vi "vision.vi"() -> ()   [LabVIEW 2024]
uses:
  <vilib>/userDefined/High Color/IMAQdx.ctl
  <vilib>/Python/Open Venv Python Session.vi
  <vilib>/vision/driver/NI_Vision_Acquisition_Software.lvlib
  <vilib>/Instr/_visa.llb/VISA Set IO Buffer Mask.ctl
  <vilib>/Instr/_visa.llb/VISA Flush IO Buffer Mask.ctl
  <vilib>/Instr/_visa.llb/VISA Configure Serial Port (Instr).vi
panel:
  in  "Serial Name":refnum<visa-resource-name>="COM1"
  out "PCU_SPEED (mps)":dbl
  out "PCU_STEER":i16
  out "PCU_ALIVE":u8
  out "하위제어기 통신 패킷":string
  out "RX Data Cnt (byte)":u32
  out "PCU_GEAR":u8
  out "PCU_MODE":u8
  out "ARD_EStop":u8
  out "PCU_ENC":i32
  in  "HLV_AorM":bool
  in  "HLV_SPEED":i16(slide) scale=0.0..1000.0
  out "TX Data Cnt (byte)":u32
  out "string":string
  in  "HLV_GEAR":u8(slide)=1 scale=0.0..2.0
  in  "HLV_EStop":bool
  out "Image":T1(plugin-control)
  in  "Session In":T2
  in  "Lane_No.":i32
  out "ToGoLane_X":dbl[](array[numeric])=[-0.07318960875272751, -0.07601258158683777, -0.07903728634119034, -0.08227015286684036, -0.08571790158748627, -0.08938748389482498, -0.09328625351190567, -0.09742185473442078, -0.1018022671341896, -0.10643591731786728, -0.11133154481649399, -0.11649835854768753, -0.12194599956274033, -0.1276845932006836, -0.13372473418712616, -0.140077605843544, -0.1467549204826355, -0.15376901626586914, -0.1611328274011612, -0.16886006295681, -0.17696507275104523, -0.18546302616596222, -0.19436998665332794, -0.20370280742645264, -0.2134794145822525, -0.22371862828731537, -0.23444052040576935, -0.2456662356853485, -0.2574182152748108, -0.26972031593322754, -0.2825978398323059, -0.2960776686668396, -0.3101884424686432, -0.3249606192111969, -0.3404266834259033, -0.35662132501602173, -0.3735816180706024, -0.39134714007377625, -0.4099603295326233, -0.4294666647911072, -0.44991496205329895, -0.47135770320892334, -0.49385130405426025, -0.5174566507339478, -0.5422393083572388, -0.5682703852653503, -0.5956265330314636, -0.6243910789489746, -0.6546544432640076, -0.6865149736404419]
  out "ToGpLane_Y":dbl[](array[numeric])=[0.040495745837688446, 0.047222185879945755, 0.05409690737724304, 0.06112465262413025, 0.06831060349941254, 0.07565993815660477, 0.08317827433347702, 0.09087134152650833, 0.09874525666236877, 0.10680633038282394, 0.1150611862540245, 0.12351679056882858, 0.13218039274215698, 0.14105971157550812, 0.1501627415418625, 0.159497931599617, 0.16907407343387604, 0.1789005994796753, 0.18898724019527435, 0.19934435188770294, 0.20998279750347137, 0.22091402113437653, 0.23215018212795258, 0.24370405077934265, 0.2555891275405884, 0.2678196132183075, 0.2804107666015625, 0.2933785319328308, 0.306739866733551, 0.3205127418041229, 0.3347163796424866, 0.349371075630188, 0.36449843645095825, 0.38012149930000305, 0.3962647616863251, 0.41295456886291504, 0.43021881580352783, 0.4480874836444855, 0.46659258008003235, 0.48576855659484863, 0.5056522488594055, 0.526283323764801, 0.5477043986320496, 0.5699615478515625, 0.5931042432785034, 0.6171862483024597, 0.6422654986381531, 0.6684049367904663, 0.6956729292869568, 0.7241437435150146]
  out "Tracking_Err(m)":dbl=0.08364582631744388
  in  "Ld(m)":dbl=1.0 format="%#_13g"
  out "GPS_Steer_CMD(Deg)":dbl=-20.0
  out "Lane":T3(graph)=[{"Third_Lane_X"=[-0.07318960875272751, -0.07601258158683777, -0.07903728634119034, -0.08227015286684036, -0.08571790158748627, -0.08938748389482498, -0.09328625351190567, -0.09742185473442078, -0.1018022671341896, -0.10643591731786728, -0.11133154481649399, -0.11649835854768753, -0.12194599956274033, -0.1276845932006836, -0.13372473418712616, -0.140077605843544, -0.1467549204826355, -0.15376901626586914, -0.1611328274011612, -0.16886006295681, -0.17696507275104523, -0.18546302616596222, -0.19436998665332794, -0.20370280742645264, -0.2134794145822525, -0.22371862828731537, -0.23444052040576935, -0.2456662356853485, -0.2574182152748108, -0.26972031593322754, -0.2825978398323059, -0.2960776686668396, -0.3101884424686432, -0.3249606192111969, -0.3404266834259033, -0.35662132501602173, -0.3735816180706024, -0.39134714007377625, -0.4099603295326233, -0.4294666647911072, -0.44991496205329895, -0.47135770320892334, -0.49385130405426025, -0.5174566507339478, -0.5422393083572388, -0.5682703852653503, -0.5956265330314636, -0.6243910789489746, -0.6546544432640076, -0.6865149736404419], "Third_Lane_Y"=[0.040495745837688446, 0.047222185879945755, 0.05409690737724304, 0.06112465262413025, 0.06831060349941254, 0.07565993815660477, 0.08317827433347702, 0.09087134152650833, 0.09874525666236877, 0.10680633038282394, 0.1150611862540245, 0.12351679056882858, 0.13218039274215698, 0.14105971157550812, 0.1501627415418625, 0.159497931599617, 0.16907407343387604, 0.1789005994796753, 0.18898724019527435, 0.19934435188770294, 0.20998279750347137, 0.22091402113437653, 0.23215018212795258, 0.24370405077934265, 0.2555891275405884, 0.2678196132183075, 0.2804107666015625, 0.2933785319328308, 0.306739866733551, 0.3205127418041229, 0.3347163796424866, 0.349371075630188, 0.36449843645095825, 0.38012149930000305, 0.3962647616863251, 0.41295456886291504, 0.43021881580352783, 0.4480874836444855, 0.46659258008003235, 0.48576855659484863, 0.5056522488594055, 0.526283323764801, 0.5477043986320496, 0.5699615478515625, 0.5931042432785034, 0.6171862483024597, 0.6422654986381531, 0.6684049367904663, 0.6956729292869568, 0.7241437435150146]}, {"Third_Lane_X"=[0.3850393295288086, 0.38269442319869995, 0.3802776634693146, 0.37778156995773315, 0.37519851326942444, 0.37252023816108704, 0.36973854899406433, 0.3668445944786072, 0.36382946372032166, 0.3606834411621094, 0.3573968708515167, 0.35395947098731995, 0.3503605127334595, 0.3465888500213623, 0.34263283014297485, 0.3384802043437958, 0.33411839604377747, 0.3295340836048126, 0.3247132897377014, 0.31964147090911865, 0.3143034875392914, 0.3086833655834198, 0.30276429653167725, 0.29652881622314453, 0.2899583876132965, 0.2830337584018707, 0.2757345139980316, 0.2680392861366272, 0.2599255442619324, 0.25136950612068176, 0.24234625697135925, 0.23282931745052338, 0.22279086709022522, 0.21220147609710693, 0.201029971241951, 0.1892433911561966, 0.17680683732032776, 0.16368332505226135, 0.14983347058296204, 0.135215625166893, 0.1197853684425354, 0.10349543392658234, 0.0862954780459404, 0.06813178956508636, 0.048946939408779144, 0.028679724782705307, 0.007264426909387112, -0.015369318425655365, -0.03929702565073967, -0.06459984183311462], "Third_Lane_Y"=[0.07649079710245132, 0.08298972249031067, 0.08961328864097595, 0.09636534750461578, 0.10325001180171967, 0.11027147620916367, 0.11743411421775818, 0.12474247813224792, 0.1322014033794403, 0.1398158222436905, 0.14759093523025513, 0.155532106757164, 0.16364507377147675, 0.17193572223186493, 0.180410236120224, 0.18907500803470612, 0.19793690741062164, 0.20700296759605408, 0.21628059446811676, 0.2257775366306305, 0.23550201952457428, 0.2454625517129898, 0.25566813349723816, 0.2661281228065491, 0.276852548122406, 0.28785181045532227, 0.29913684725761414, 0.31071919202804565, 0.32261112332344055, 0.33482545614242554, 0.3473757207393646, 0.3602762222290039, 0.3735422194004059, 0.387189656496048, 0.4012354910373688, 0.4156976342201233, 0.4305952489376068, 0.4459485411643982, 0.4617789089679718, 0.4781092703342438, 0.4949638843536377, 0.5123687386512756, 0.5303513407707214, 0.5489413142204285, 0.5681700706481934, 0.5880714654922485, 0.6086814403533936, 0.6300389170646667, 0.6521854400634766, 0.6751657128334045]}, {"Third_Lane_X"=[0.0, 0.0, 0.0, 0.0, 0.0, 0.0, 0.0, 0.0, 0.0, 0.0, 0.0, 0.0, 0.0, 0.0, 0.0, 0.0, 0.0, 0.0, 0.0, 0.0, 0.0, 0.0, 0.0, 0.0, 0.0, 0.0, 0.0, 0.0, 0.0, 0.0, 0.0, 0.0, 0.0, 0.0, 0.0, 0.0, 0.0, 0.0, 0.0, 0.0, 0.0, 0.0, 0.0, 0.0, 0.0, 0.0, 0.0, 0.0, 0.0, 0.0], "Third_Lane_Y"=[0.0, 0.0, 0.0, 0.0, 0.0, 0.0, 0.0, 0.0, 0.0, 0.0, 0.0, 0.0, 0.0, 0.0, 0.0, 0.0, 0.0, 0.0, 0.0, 0.0, 0.0, 0.0, 0.0, 0.0, 0.0, 0.0, 0.0, 0.0, 0.0, 0.0, 0.0, 0.0, 0.0, 0.0, 0.0, 0.0, 0.0, 0.0, 0.0, 0.0, 0.0, 0.0, 0.0, 0.0, 0.0, 0.0, 0.0, 0.0, 0.0, 0.0]}]
  out "Third_Lane_X":dbl[](array[numeric])
  out "Third_Lane_Y":dbl[](array[numeric])
  out "Second_Lane_X":dbl[](array[numeric])=[0.3850393295288086, 0.38269442319869995, 0.3802776634693146, 0.37778156995773315, 0.37519851326942444, 0.37252023816108704, 0.36973854899406433, 0.3668445944786072, 0.36382946372032166, 0.3606834411621094, 0.3573968708515167, 0.35395947098731995, 0.3503605127334595, 0.3465888500213623, 0.34263283014297485, 0.3384802043437958, 0.33411839604377747, 0.3295340836048126, 0.3247132897377014, 0.31964147090911865, 0.3143034875392914, 0.3086833655834198, 0.30276429653167725, 0.29652881622314453, 0.2899583876132965, 0.2830337584018707, 0.2757345139980316, 0.2680392861366272, 0.2599255442619324, 0.25136950612068176, 0.24234625697135925, 0.23282931745052338, 0.22279086709022522, 0.21220147609710693, 0.201029971241951, 0.1892433911561966, 0.17680683732032776, 0.16368332505226135, 0.14983347058296204, 0.135215625166893, 0.1197853684425354, 0.10349543392658234, 0.0862954780459404, 0.06813178956508636, 0.048946939408779144, 0.028679724782705307, 0.007264426909387112, -0.015369318425655365, -0.03929702565073967, -0.06459984183311462]
  out "Second_Lane_Y":dbl[](array[numeric])=[0.07649079710245132, 0.08298972249031067, 0.08961328864097595, 0.09636534750461578, 0.10325001180171967, 0.11027147620916367, 0.11743411421775818, 0.12474247813224792, 0.1322014033794403, 0.1398158222436905, 0.14759093523025513, 0.155532106757164, 0.16364507377147675, 0.17193572223186493, 0.180410236120224, 0.18907500803470612, 0.19793690741062164, 0.20700296759605408, 0.21628059446811676, 0.2257775366306305, 0.23550201952457428, 0.2454625517129898, 0.25566813349723816, 0.2661281228065491, 0.276852548122406, 0.28785181045532227, 0.29913684725761414, 0.31071919202804565, 0.32261112332344055, 0.33482545614242554, 0.3473757207393646, 0.3602762222290039, 0.3735422194004059, 0.387189656496048, 0.4012354910373688, 0.4156976342201233, 0.4305952489376068, 0.4459485411643982, 0.4617789089679718, 0.4781092703342438, 0.4949638843536377, 0.5123687386512756, 0.5303513407707214, 0.5489413142204285, 0.5681700706481934, 0.5880714654922485, 0.6086814403533936, 0.6300389170646667, 0.6521854400634766, 0.6751657128334045]
  out "First_Lane_Y":dbl[](array[numeric])=[0.040495745837688446, 0.047222185879945755, 0.05409690737724304, 0.06112465262413025, 0.06831060349941254, 0.07565993815660477, 0.08317827433347702, 0.09087134152650833, 0.09874525666236877, 0.10680633038282394, 0.1150611862540245, 0.12351679056882858, 0.13218039274215698, 0.14105971157550812, 0.1501627415418625, 0.159497931599617, 0.16907407343387604, 0.1789005994796753, 0.18898724019527435, 0.19934435188770294, 0.20998279750347137, 0.22091402113437653, 0.23215018212795258, 0.24370405077934265, 0.2555891275405884, 0.2678196132183075, 0.2804107666015625, 0.2933785319328308, 0.306739866733551, 0.3205127418041229, 0.3347163796424866, 0.349371075630188, 0.36449843645095825, 0.38012149930000305, 0.3962647616863251, 0.41295456886291504, 0.43021881580352783, 0.4480874836444855, 0.46659258008003235, 0.48576855659484863, 0.5056522488594055, 0.526283323764801, 0.5477043986320496, 0.5699615478515625, 0.5931042432785034, 0.6171862483024597, 0.6422654986381531, 0.6684049367904663, 0.6956729292869568, 0.7241437435150146]
  out "First_Lane_X":dbl[](array[numeric])=[-0.07318960875272751, -0.07601258158683777, -0.07903728634119034, -0.08227015286684036, -0.08571790158748627, -0.08938748389482498, -0.09328625351190567, -0.09742185473442078, -0.1018022671341896, -0.10643591731786728, -0.11133154481649399, -0.11649835854768753, -0.12194599956274033, -0.1276845932006836, -0.13372473418712616, -0.140077605843544, -0.1467549204826355, -0.15376901626586914, -0.1611328274011612, -0.16886006295681, -0.17696507275104523, -0.18546302616596222, -0.19436998665332794, -0.20370280742645264, -0.2134794145822525, -0.22371862828731537, -0.23444052040576935, -0.2456662356853485, -0.2574182152748108, -0.26972031593322754, -0.2825978398323059, -0.2960776686668396, -0.3101884424686432, -0.3249606192111969, -0.3404266834259033, -0.35662132501602173, -0.3735816180706024, -0.39134714007377625, -0.4099603295326233, -0.4294666647911072, -0.44991496205329895, -0.47135770320892334, -0.49385130405426025, -0.5174566507339478, -0.5422393083572388, -0.5682703852653503, -0.5956265330314636, -0.6243910789489746, -0.6546544432640076, -0.6865149736404419]
  out "error out":errorcluster
  out "Python Loop Process Time":u32=34
  in  "stop":bool
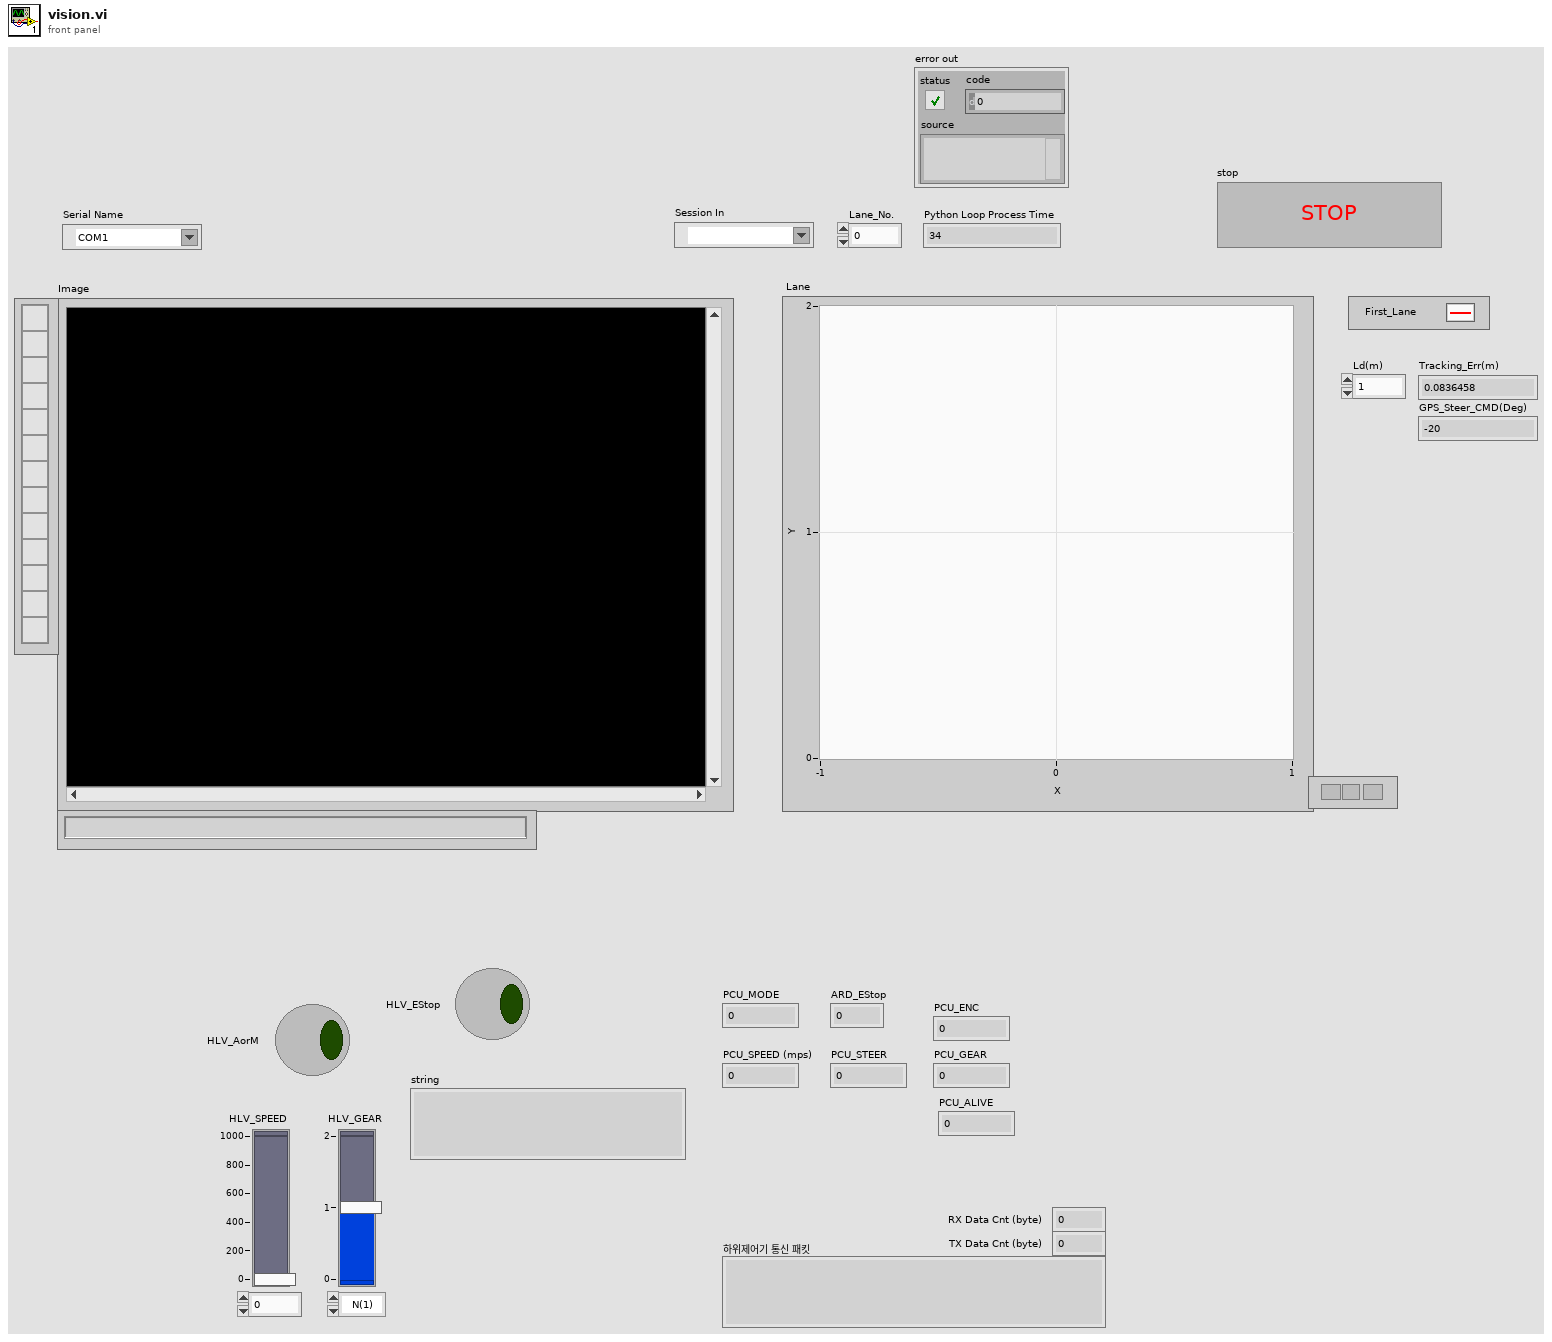
[diagram p1: front panel]
types:
  T1 = typedef "IMAQ Image.ctl" = refnum<image>
  T2 = typedef "IMAQdx.ctl" = refnum<k21>
  T3 = cluster{"Third_Lane_X":dbl[], "Third_Lane_Y":dbl[]}[]
  T4 = cluster{"HLV_M/A_Status":u8, "HLV_EStop":u8, "HLV_Gear":u8, "HLV_Speed":i16, "HLV_Steer":i16, "HLV_Alive":u8}
  T5 = cluster{"ARD_M/A_Status":u8, "ARD_EStop":u8, "ARD_Gear":u8, "ARD_Speed":i16, "ARD_Steer":i16, "ARD_ENC":i32, "ARD_Alive":u8}
  T6 = typedef "VISA Flush IO Buffer Mask.ctl" = u16
  T7 = typedef "VISA Set IO Buffer Mask.ctl" = u16
  T8 = cluster{"First_Lane_X":dbl[], "First_Lane_Y":dbl[]}
  T9 = cluster{"Second_Lane_X":dbl[], "Second_Lane_Y":dbl[]}
  T10 = cluster{"Third_Lane_X":dbl[], "Third_Lane_Y":dbl[]}
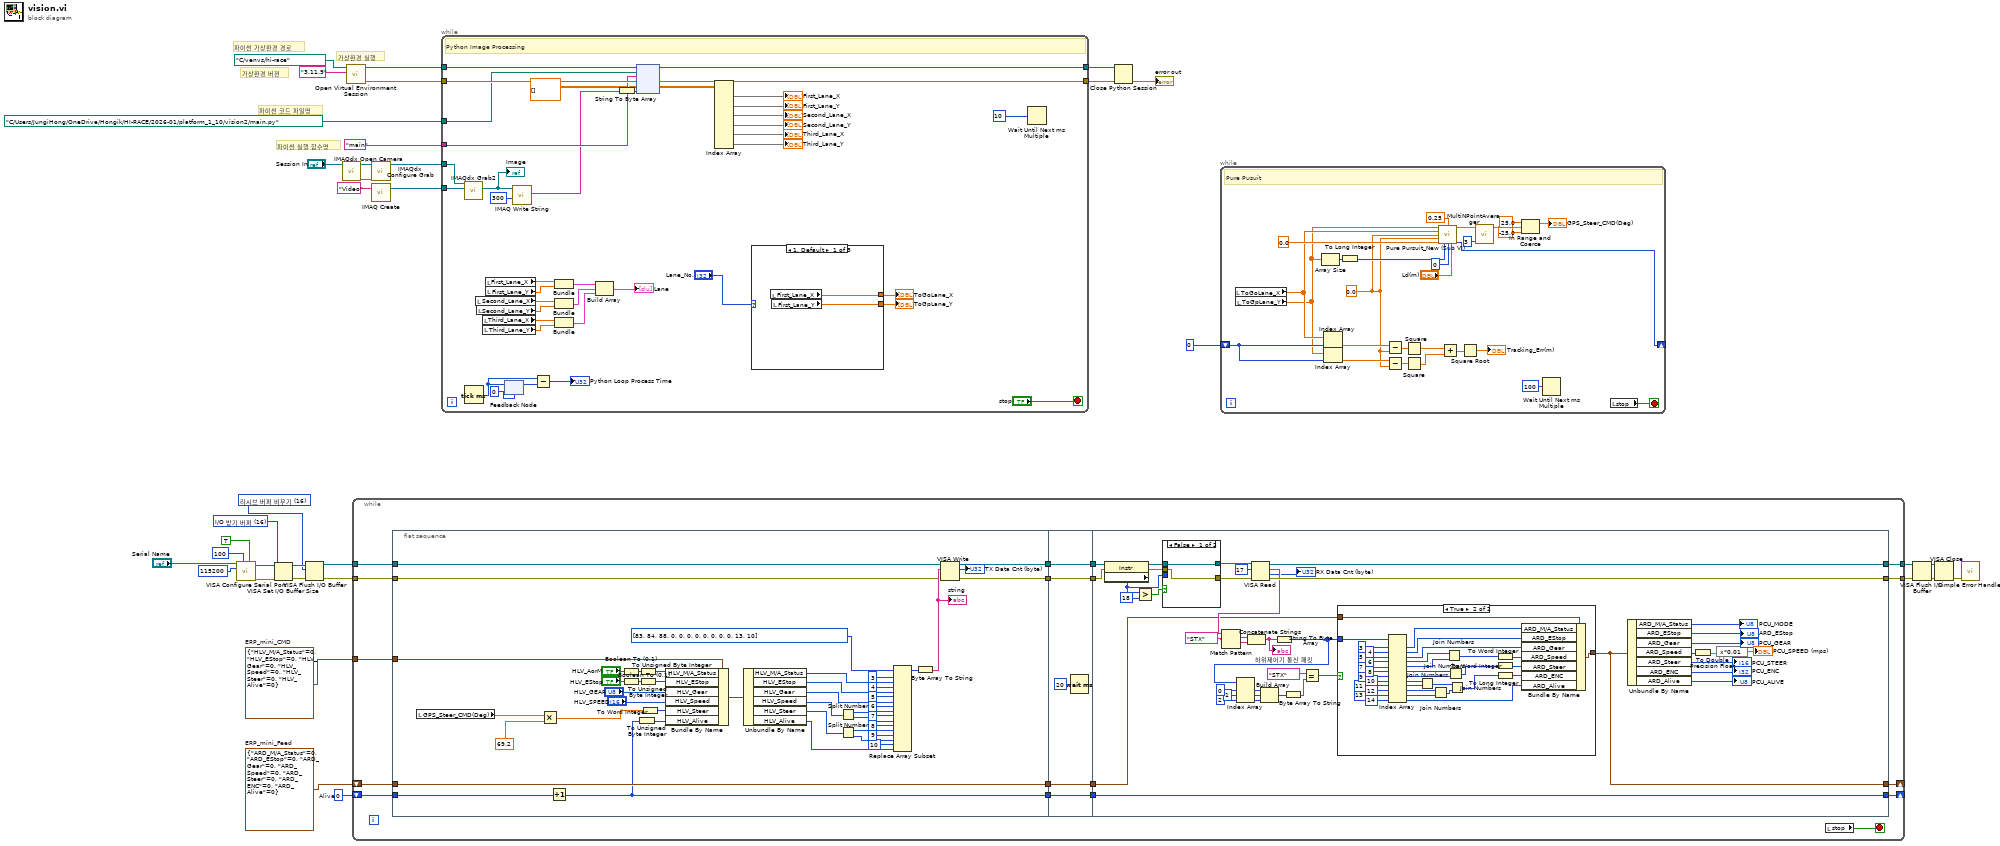
[diagram p0: block diagram]
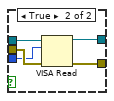
[diagram p2: hidden frame]
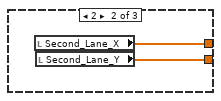
[diagram p4: hidden frame]
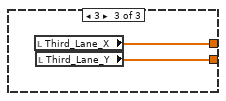
[diagram p5: hidden frame]
diagram:
  w13 = T4 {"HLV_M/A_Status"=0, "HLV_EStop"=0, "HLV_Gear"=0, "HLV_Speed"=0, "HLV_Steer"=0, "HLV_Alive"=0}  # ERP_mini_CMD
  w14 = T5 {"ARD_M/A_Status"=0, "ARD_EStop"=0, "ARD_Gear"=0, "ARD_Speed"=0, "ARD_Steer"=0, "ARD_ENC"=0, "ARD_Alive"=0}  # ERP_mini_Feed
  w1 = u8 0  # Alive
  w4 = T6 16 items=["리시브 버퍼 비우기"=16, "전달 버퍼 디바이스에 쓰기"=32, "리시브 버퍼 비우기(I/O 없음)"=64, "전달 버퍼 비우기"=128] ("Mask")
  w7 = T7 16 items=["I/O 받기 버퍼"=16, "I/O 전달 버퍼"=32, "I/O 받기와 전달 버퍼"=48] ("Mask")
  # "파이썬 실행 함수명"
  # "파이썬 코드 파일명"
  # "가상환경 실행"
  # "가상환경 버젼"
  # "파이썬 가상환경 경로"
  n1 = call-poly "VISA Configure Serial Port"("VISA resource name"="Serial Name", "timeout (10sec)"=u32 100, "Enable Termination\nChar (T)"=TRUE ("Enable Termination\nChar (T)"), "baud rate (9600)"=u32 115200) -> ("VISA resource name out"=w9:refnum<visa-resource-name>, "error out"=w8:errorcluster)  [unwired: 10 in]
  n2 = VISA Set I/O Buffer Size(VISA resource name=w9, mask (16)=w7, error in (no error)=w8) -> (VISA resource name out=w6:refnum<visa-resource-name>, error out=w5:errorcluster)  [unwired: 1 in]
  n3 = VISA Flush I/O Buffer(VISA resource name=w6, mask (16)=w4, error in (no error)=w5) -> (VISA resource name out=w18:refnum<visa-resource-name>, error out=w2:errorcluster)
  n4 = call <vilib>:"IMAQdx Open Camera.vi"("Session In"="Session In") -> ("error out"=w24:errorcluster, "Session Out"=w23:T2)  [unwired: 9 in]
  n5 = call-poly <vilib>:"Open Virtual Environment Session.vi"("Python version"="3.11.9", "Env path"=path "C:/venvs/hi-race") -> ("error out"=w31:errorcluster, "session out"=w32:refnum<k35>)  [unwired: 8 in]
  n6 = while {
    tunnel: w18 -> [w54]
    tunnel: w2 -> [w53]
    tunnel: [w48] -> w17
    tunnel: [w47] -> w16
    shift-right: [w43] -> _
    shift-left: w14 -> [w45]
    tunnel: w13 -> [w42]
    shift-right: [w38] -> _
    shift-left: w1 -> [w41]
    stop <- w37 stop-if-true
    n7 = flat-sequence {
      tunnel: [w84] -> w51
      tunnel: [w83] -> w49
      tunnel: w54 -> [w86]
      tunnel: w53 -> [w85]
      tunnel: [w81] -> w46
      tunnel: w45 -> [w81]
      tunnel: w42 -> [w80]
      tunnel: w41 -> [w77]
      tunnel: [w76] -> w39
      tunnel: [w103] -> w52
      tunnel: w51 -> [w103]
      tunnel: [w102] -> w50
      tunnel: w49 -> [w102]
      tunnel: w46 -> [w101]
      tunnel: [w101] -> w44
      tunnel: [w100] -> w40
      tunnel: w39 -> [w100]
      tunnel: w52 -> [w122]
      tunnel: w50 -> [w121]
      tunnel: [w144] -> w48
      tunnel: [w143] -> w47
      tunnel: w44 -> [w124]
      tunnel: [w123] -> w43
      tunnel: [w113] -> w38
      tunnel: w40 -> [w113]
      frame #0 {
        n8 = local read "GPS_Steer_CMD(Deg)"() -> (w57:dbl)
        n9 = Multiply(x=w57, y=69.2) -> (x*y=w55:dbl)
        n10 = Increment(x=w77) -> (x+1=w76:u8)
        n11 = Boolean To (0,1)(Boolean="HLV_AorM") -> (0, 1=w78:i16)
        n12 = Boolean To (0,1)(Boolean="HLV_EStop") -> (0, 1=w69:i16)
        n13 = To Unsigned Byte Integer(number=w76) -> (unsigned 8bit integer=w92:u8)
        n14 = To Unsigned Byte Integer(number=w78) -> (unsigned 8bit integer=w70:u8)
        n15 = To Unsigned Byte Integer(number=w69) -> (unsigned 8bit integer=w67:u8)
        n16 = To Word Integer(number=w55) -> (16bit integer=w79:i16)
        n17 = Bundle By Name(cluster=w80, "HLV_M/A_Status"=w70, "HLV_EStop"=w67, "HLV_Gear"="HLV_GEAR", "HLV_Speed"="HLV_SPEED", "HLV_Steer"=w79, "HLV_Alive"=w92) -> (w87:T4)
        n18 = Unbundle By Name(w87) -> ("HLV_M/A_Status"=w66:u8, "HLV_EStop"=w65:u8, "HLV_Gear"=w64:u8, "HLV_Speed"=w72:i16, "HLV_Steer"=w71:i16, "HLV_Alive"=w58:u8)
        n19 = Split Number(x=w72) -> (hi(x)=w63:u8, lo(x)=w62:u8)
        n20 = Split Number(x=w71) -> (hi(x)=w61:u8, lo(x)=w60:u8)
        n21 = Replace Array Subset(array=u8[] [83, 84, 88, 0, 0, 0, 0, 0, 0, 0, 0, 13, 10] ("unsigned byte array"), new element #1=w66, index #1=3, new element #2=w65, index #2=4, new element #3=w64, index #3=5, new element #4=w63, index #4=6, new element #5=w62, index #5=7, new element #6=w61, index #6=8, new element #7=w60, index #7=9, new element #8=w58, index #8=10) -> (w96:u8[])
        n22 = Byte Array To String(unsigned byte array=w96) -> (string=w97:string)
        "string" <- w97
        n23 = VISA Write(VISA resource name=w86, write buffer=w97, error in (no error)=w85) -> (VISA resource name out=w84:refnum<visa-resource-name>, return count=→"TX Data Cnt (byte)":u32, error out=w83:errorcluster)
      }
      frame #1 {
        n24 = Wait (ms)(milliseconds to wait=u32 20 ("대기 시간 (ms)")) -> ()  [unwired: 1 out]
      }
      frame #2 {
        n25 = property class="Instr"(reference=w122, error in=w121) -> (reference out=w120:refnum<visa-resource-name>, error out=w119:errorcluster, "Serial Settings:Number of Bytes at Serial Port"=w114:u32)
        n26 = Greater?(x=w114, y=u32 18) -> (0:w116:bool)
        n27 = case shown="False" w116 {
          tunnel: w120 -> [w146 w151]
          tunnel: w119 -> [w145 w150]
          tunnel: [w146 w149] -> w118
          tunnel: [w145 w148] -> w117
          tunnel: w114 -> [_ w147]
          frame False {
          }
          frame True {
            n28 = VISA Read(VISA resource name=w151, byte count=w147, error in (no error)=w150) -> (VISA resource name out=w149:refnum<visa-resource-name>, error out=w148:errorcluster)  [unwired: 2 out]
          }
        }
        n29 = VISA Read(VISA resource name=w118, byte count=u32 17, error in (no error)=w117) -> (VISA resource name out=w144:refnum<visa-resource-name>, read buffer=w142:string, return count=→"RX Data Cnt (byte)":u32, error out=w143:errorcluster)
        n30 = Match Pattern(string=w142, regular expression="STX") -> (match substring=w139:string, after substring=w140:string)  [unwired: 1 in, 2 out]
        n31 = Concatenate Strings(w139, w140) -> (w138:string)
        "하위제어기 통신 패킷" <- w138
        n32 = String To Byte Array(string=w138) -> (unsigned byte array=w126:u8[])
        n33 = Index Array(array=w126, index #1=0, index #2=1, index #3=2) -> (element #1=w132:u8, element #2=w131:u8, element #3=w130:u8)
        n34 = Build Array(w132, w131, w130) -> (w129:u8[])
        n35 = Byte Array To String(unsigned byte array=w129) -> (string=w127:string)
        n36 = Equal?(x="STX", y=w127) -> (x = y?=w125:bool)
        n37 = case shown="True" w125 {
          tunnel: w126 -> [_ w187]
          tunnel: [w152 w186] -> w123
          tunnel: w124 -> [w152 w185]
          frame False {
          }
          frame True {
            n38 = Index Array(array=w187, index #1=3, index #2=4, index #3=5, index #4=6, index #5=7, index #6=8, index #7=9, index #8=10, index #9=11, index #10=12, index #11=13, index #12=14) -> (element #1=w174:u8, element #2=w173:u8, element #3=w172:u8, element #4=w171:u8, element #5=w170:u8, element #6=w168:u8, element #7=w167:u8, element #8=w159:u8, element #9=w158:u8, element #10=w157:u8, element #11=w156:u8, element #12=w161:u8)
            n39 = Join Numbers(hi=w159, lo=w158) -> ((hi.lo)=w155:u16)
            n40 = Join Numbers(hi=w157, lo=w156) -> ((hi.lo)=w154:u16)
            n41 = Join Numbers(hi=w171, lo=w170) -> ((hi.lo)=w169:u16)
            n42 = Join Numbers(hi=w168, lo=w167) -> ((hi.lo)=w166:u16)
            n43 = Join Numbers(hi=w155, lo=w154) -> ((hi.lo)=w153:u32)
            n44 = To Word Integer(number=w169) -> (16bit integer=w178:i16)
            n45 = To Word Integer(number=w166) -> (16bit integer=w177:i16)
            n46 = To Long Integer(number=w153) -> (32bit integer=w160:i32)
            n47 = Bundle By Name(cluster=w185, "ARD_M/A_Status"=w174, "ARD_EStop"=w173, "ARD_Gear"=w172, "ARD_Speed"=w178, "ARD_Steer"=w177, "ARD_ENC"=w160, "ARD_Alive"=w161) -> (w186:T5)
          }
        }
        n48 = Unbundle By Name(w123) -> ("ARD_M/A_Status"=→"PCU_MODE":u8, "ARD_EStop"=→"ARD_EStop":u8, "ARD_Gear"=→"PCU_GEAR":u8, "ARD_Speed"=w110:i16, "ARD_Steer"=→"PCU_STEER":i16, "ARD_ENC"=→"PCU_ENC":i32, "ARD_Alive"=→"PCU_ALIVE":u8)
        n49 = To Double Precision Float(number=w110) -> (double precision float=w111:dbl)
        n50 = expression code="x*0.01"(w111) -> (→"PCU_SPEED (mps)":dbl)
      }
    }
    n51 = local read "stop"() -> (w37:bool)
  }
  n52 = call <vilib>:"IMAQdx Configure Grab.vi"("error in"=w24, "Session In"=w23) -> ("Session Out"=w22:T2)  [unwired: 8 in, 1 out]
  n53 = call "IMAQ Create"("Image Name"="Video") -> ("New Image"=w25:T1)  [unwired: 4 in, 1 out]
  n54 = while {
    tunnel: path "C:/Users/JungiHong/OneDrive/Hongik/HI-RACE/2026-01/platform_1_10/vision2/main.py" ("Name") -> [w222]
    tunnel: "main" ("module out") -> [w221]
    tunnel: w32 -> [w224]
    tunnel: [w226] -> w34
    tunnel: w31 -> [w223]
    tunnel: [w225] -> w33
    tunnel: w25 -> [w190]
    tunnel: w22 -> [w189]
    stop <- "stop" stop-if-true
    # "Python Image Processing"
    n55 = call <vilib>:"IMAQdx Grab2.vi"("Image In"=w190, "Session In"=w189) -> ("Image Out"=w188:T1)  [unwired: 6 in, 3 out]
    "Image" <- w188
    n56 = Tick Count (ms)() -> (millisecond timer value=w217:u32)
    n57 = local read "Second_Lane_X"() -> (w207:dbl[])
    n58 = local read "Second_Lane_Y"() -> (w206:dbl[])
    n59 = local read "Third_Lane_X"() -> (w205:dbl[])
    n60 = local read "Third_Lane_Y"() -> (w204:dbl[])
    n61 = local read "First_Lane_X"() -> (w209:dbl[])
    n62 = local read "First_Lane_Y"() -> (w208:dbl[])
    n63 = feedback #1(u32 0 ("millisecond timer value")) -> (w218:u32)
    n64 = feedback-in #1(w217) -> ()
    n65 = call-poly "IMAQ Write String"("Image Quality"=u32 300, "Image"=w188) -> ("FileString"=w191:string)  [unwired: 7 in, 2 out]
    n66 = Subtract(x=w217, y=w218) -> (x-y=→"Python Loop Process Time":u32)
    n67 = Bundle("First_Lane_X"=w209, "First_Lane_Y"=w208) -> (w203:T8)  [unwired: 1 in]
    n68 = Bundle("Second_Lane_X"=w207, "Second_Lane_Y"=w206) -> (w202:T9)  [unwired: 1 in]
    n69 = Bundle("Third_Lane_X"=w205, "Third_Lane_Y"=w204) -> (w201:T10)  [unwired: 1 in]
    n70 = Build Array(w203, w202, w201) -> (→"Lane":T3)
    n71 = String To Byte Array(string=w191) -> (unsigned byte array=w216:u8[])
    n72 = node(w224, w222, w221, w223, dbl[][] [] ("appended array"), w216) -> (w226:refnum<k35>, w225:errorcluster, w195:dbl[][])  [unwired: 1 in, 2 out]
    n73 = Index Array(array=w195) -> (element #1=→"First_Lane_X":dbl[], element #2=→"First_Lane_Y":dbl[], element #3=→"Second_Lane_X":dbl[], element #4=→"Second_Lane_Y":dbl[], element #5=→"Third_Lane_X":dbl[], element #6=→"Third_Lane_Y":dbl[])  [unwired: 12 in]
    n74 = case shown="1, Default" "Lane_No." {
      tunnel: [w228 w230 w232] -> w198
      tunnel: [w227 w229 w231] -> w197
      frame 1, Default {
        n75 = local read "First_Lane_X"() -> (w228:dbl[])
        n76 = local read "First_Lane_Y"() -> (w227:dbl[])
      }
      frame 2 {
        n77 = local read "Second_Lane_X"() -> (w230:dbl[])
        n78 = local read "Second_Lane_Y"() -> (w229:dbl[])
      }
      frame 3 {
        n79 = local read "Third_Lane_X"() -> (w232:dbl[])
        n80 = local read "Third_Lane_Y"() -> (w231:dbl[])
      }
    }
    "ToGoLane_X" <- w198
    "ToGpLane_Y" <- w197
    n81 = Wait Until Next ms Multiple(millisecond multiple=u32 10) -> ()  [unwired: 1 out]
  }
  n82 = Close Python Session(session in=w34, error in=w33) -> (11:→"error out":errorcluster)
  n83 = while {
    shift-right: [w259] -> _
    shift-left: 0 ("Index(near vehicle)") -> [w258]
    stop <- w257 stop-if-true
    w233 = 0.0 ("Y_Current")
    # "Pure Pusuit"
    n84 = local read "ToGoLane_X"() -> (w235:dbl[])
    n85 = local read "ToGpLane_Y"() -> (w234:dbl[])
    n86 = Array Size(array=w234) -> (size(s)=w244:i32)
    n87 = Index Array(array=w235, index=w258) -> (element=w255:dbl)
    n88 = Index Array(array=w234, index=w258) -> (element=w256:dbl)
    n89 = To Long Integer(number=w244) -> (32bit integer=w243:i32)
    n90 = Subtract(x=w255, y=w233) -> (x-y=w250:dbl)
    n91 = Subtract(x=w256, y=w233) -> (x-y=w249:dbl)
    n92 = Square(x=w250) -> (x^2=w248:dbl)
    n93 = Square(x=w249) -> (x^2=w247:dbl)
    n94 = call "Pure Pursuit_New (Sub VI).vi"("x_lat_path"=w234, "L"=0.25, "y_long_path"=w235, "X_Current"=w233, "Y_Current"=w233, "Heading_Current"=0.0, "#pnt"=w243, "WP no_pre"=0, "LAD"="Ld(m)") -> ("Steer_CMD(Deg)"=w239:dbl, "Index(near vehicle)"=w259:i32)  [unwired: 3 in, 2 out]
    n95 = Add(x=w248, y=w247) -> (x+y=w246:dbl)
    n96 = Square Root(x=w246) -> (sqrt(x)=→"Tracking_Err(m)":dbl)
    n97 = call "MultiNPointAverager.vi"("N point average"=3 ("WP no_pre"), "Data_input"=w239) -> ("숫자형"=w254:dbl)  [unwired: 9 in]
    n98 = In Range and Coerce(upper limit=25.0, x=w254, lower limit=-25.0) -> (coerced(x)=→"GPS_Steer_CMD(Deg)":dbl)  [unwired: 1 out]
    n99 = Wait Until Next ms Multiple(millisecond multiple=u32 100 ("ms 배수")) -> ()  [unwired: 1 out]
    n100 = local read "stop"() -> (w257:bool)
  }
  n101 = VISA Flush I/O Buffer(VISA resource name=w17, error in (no error)=w16) -> (VISA resource name out=w19:refnum<visa-resource-name>, error out=w20:errorcluster)  [unwired: 1 in]
  n102 = VISA Close(VISA resource name=w19, error in (no error)=w20) -> (error out=w15:errorcluster)
  n103 = call <vilib>:"Simple Error Handler.vi"("error in (no error)"=w15) -> ()  [unwired: 4 in, 5 out]
